vi "Own20261012_SetInvokeClass.vi"() -> ()   [LabVIEW 2024]
panel:
  out "error out":errorcluster caption="错误输出"
  in  "class_name":string
  in  "invoke_id":u32
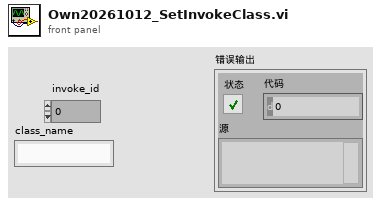
[diagram p1: front panel]
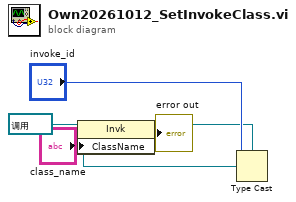
[diagram p0: block diagram]
diagram:
  n1 = Type Cast(type=refnum<vi> refnum ("引用"), x="invoke_id") -> (*(type *) &x=w3:refnum<vi>)
  n2 = property class="Invk"(reference=w3, "ClassName"="class_name") -> (error out=→"error out":errorcluster)  [unwired: 1 in, 1 out]
